vi "Register Events.vi"(8 "error in (no error)":errorcluster, 11 "WebView2 Control in":refnum<class "WebView2 Control.lvclass">) -> (0 "error out":errorcluster, 2 "Events":T1, 3 "WebView2 Control out":refnum<class "WebView2 Control.lvclass">)   [LabVIEW 2020, in "WebView2.lvlib" / "WebView2 Control.lvclass"]
uses:
  WebView2 Control.lvclass
  WebView2 Event Filter Interface/WebView2 Event Filter Interface.lvclass
  E:/Labview/LV 2023/PPL/PPL Builder/Libs/LV-WebView2/Source/Libs/Microsoft.Web.WebView2.Core.dll
  Libs/Microsoft.Web.WebView2.Core.dll
  WebView2 Control.lvclass/WebView2 Control.ctl
  _Raise Nav Complete Event.vi
  _Raise Navigation Starting Event.vi
  _Raise Source Changed Event.vi
  _Raise Document Title Changed.vi
  _Raise StatusBarTextChanged.vi
  _Raise WebMessageReceived.vi
  _Raise WindowCloseRequested.vi
  _Raise Dom Content Loaded.vi
  _Raise New Window Requested.vi
  _Raise Content Loading.vi
  _Raise Context Menu Requested.vi
  _Raise Download Starting.vi
  _Raise Favicon Changed.vi
  _Raise Launching External Uri Scheme.vi
  _Raise Notification Received.vi
  _Raise Permission Requested.vi
  _Raise Save As UI Showing.vi
  _Raise Save File Security Check Starting.vi
  _Raise Script Dialog Opening.vi
  _Raise Server Certificate Error Detected.vi
  _Raise Basic Authentication Requested.vi
  _Raise Client Certificate Requested.vi
  Navigation Event Data.ctl
  Source Changed Event Data.ctl
  Navigation Start Event Data.ctl
  Events.ctl
  New Window Event Data.ctl
  Content Loading Event Data.ctl
  Web Message Received Event Data.ctl
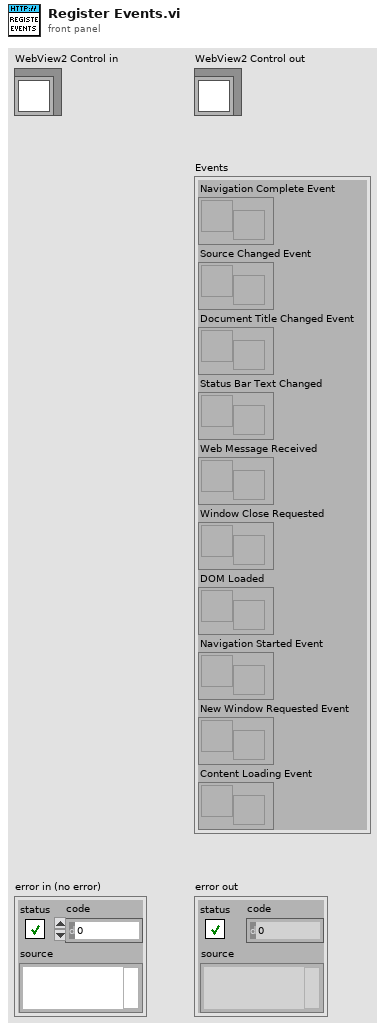
[diagram p1: front panel]
types:
  T1 = typedef "WebView2.lvlib/WebView2 Control.lvclass/Events.ctl" = cluster{"Navigation Complete Event":refnum<user-event>, "Source Changed Event":refnum<user-event>, "Document Title Changed Event":refnum<user-event>, "Status Bar Text Changed":refnum<user-event>, "Web Message Received":refnum<user-event>, "Window Close Requested":refnum<user-event>, "DOM Loaded":refnum<user-event>, "Navigation Started Event":refnum<user-event>, "New Window Requested Event":refnum<user-event>, "Content Loading Event":refnum<user-event>}
  T2 = typedef "WebView2.lvlib/WebView2 Control.lvclass/Res.ctl" = cluster{"WebView2":refnum<k24>, "Webview2 Core":refnum<k24>, "event callback":refnum<k27>, "Environment":refnum<k24>}
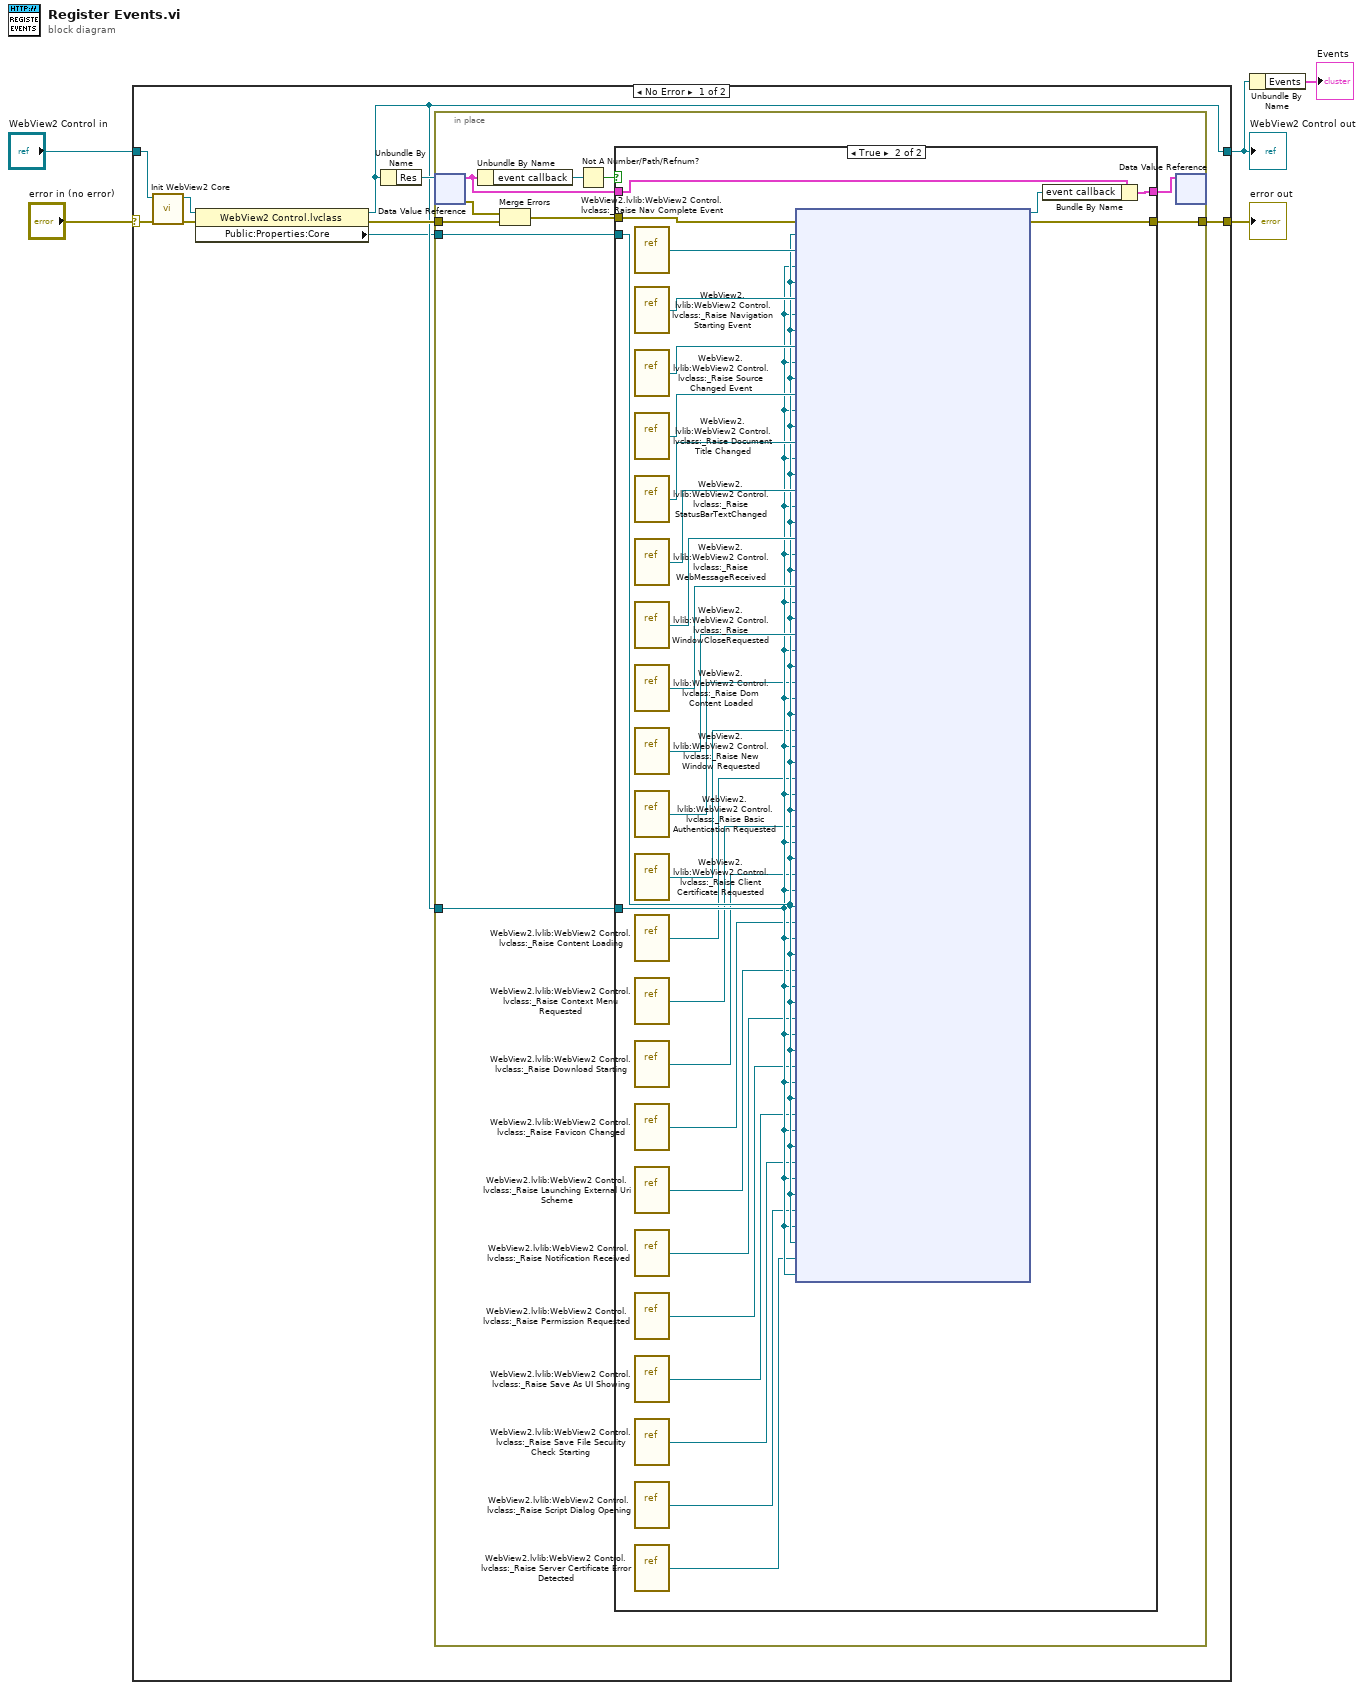
[diagram p0: block diagram]
diagram:
  n1 = case shown="No Error" "error in (no error)" {
    selector: "error in (no error)" -> [w13 w57]
    tunnel: [w7 w56] -> w1
    tunnel: "WebView2 Control in" -> [w14 w56]
    tunnel: [w10 w57] -> w3
    frame No Error {
      n2 = call "Init WebView2 Core.vi"("error in (no error)"=w13, "WebView2"=w14) -> ("error out"=w11:errorcluster, "WebView2.lvlib:WebView2 Control.lvclass"=w8:refnum<class "WebView2 Control.lvclass">)  [unwired: 8 in]
      n3 = property class="WebView2 Control.lvclass"(reference=w8, error in=w11) -> (reference out=w7:refnum<class "WebView2 Control.lvclass">, error out=w9:errorcluster, "Public:Properties:Core"=w6:refnum<k24>)
      n4 = Unbundle By Name(w7) -> ("Res"=w12:refnum<data-value>)
      n5 = in-place {
        in-place-border: w9 -> [w24]
        in-place-border: w7 -> [w21]
        in-place-border: [w20] -> w10
        in-place-border: w6 -> [w15]
        n6 = in-place-dvr #1(w12) -> (w17:T2, w23:errorcluster)
        n7 = Unbundle By Name(w17) -> ("event callback"=w19:refnum<k27>)
        n8 = Merge Errors(w23, w24) -> (w22:errorcluster)
        n9 = Not A Number/Path/Refnum?(number/path/refnum=w19) -> (NaN/Path/Refnum?=w18:bool)
        n10 = case shown="True" w18 {
          tunnel: [w26 w55] -> w20
          tunnel: w22 -> [w26 w51]
          tunnel: w21 -> [_ w40]
          tunnel: w17 -> [w25 w52]
          tunnel: [w25 w53] -> w16
          tunnel: w15 -> [_ w41]
          frame False {
          }
          frame True {
            n11 = vi-ref "WebView2.lvlib:WebView2 Control.lvclass:_Raise Nav Complete Event.vi"() -> (w50:refnum<vi>)
            n12 = vi-ref "WebView2.lvlib:WebView2 Control.lvclass:_Raise Navigation Starting Event.vi"() -> (w49:refnum<vi>)
            n13 = vi-ref "WebView2.lvlib:WebView2 Control.lvclass:_Raise Source Changed Event.vi"() -> (w48:refnum<vi>)
            n14 = vi-ref "WebView2.lvlib:WebView2 Control.lvclass:_Raise Document Title Changed.vi"() -> (w47:refnum<vi>)
            n15 = vi-ref "WebView2.lvlib:WebView2 Control.lvclass:_Raise StatusBarTextChanged.vi"() -> (w46:refnum<vi>)
            n16 = vi-ref "WebView2.lvlib:WebView2 Control.lvclass:_Raise WebMessageReceived.vi"() -> (w45:refnum<vi>)
            n17 = vi-ref "WebView2.lvlib:WebView2 Control.lvclass:_Raise WindowCloseRequested.vi"() -> (w44:refnum<vi>)
            n18 = vi-ref "WebView2.lvlib:WebView2 Control.lvclass:_Raise Dom Content Loaded.vi"() -> (w43:refnum<vi>)
            n19 = vi-ref "WebView2.lvlib:WebView2 Control.lvclass:_Raise New Window Requested.vi"() -> ("vi reference"=w42:refnum<vi>)
            n20 = vi-ref "WebView2.lvlib:WebView2 Control.lvclass:_Raise Basic Authentication Requested.vi"() -> ("vi reference"=w28:refnum<vi>)
            n21 = vi-ref "WebView2.lvlib:WebView2 Control.lvclass:_Raise Client Certificate Requested.vi"() -> ("vi reference"=w27:refnum<vi>)
            n22 = vi-ref "WebView2.lvlib:WebView2 Control.lvclass:_Raise Content Loading.vi"() -> ("vi reference"=w39:refnum<vi>)
            n23 = vi-ref "WebView2.lvlib:WebView2 Control.lvclass:_Raise Context Menu Requested.vi"() -> ("vi reference"=w38:refnum<vi>)
            n24 = vi-ref "WebView2.lvlib:WebView2 Control.lvclass:_Raise Download Starting.vi"() -> ("vi reference"=w37:refnum<vi>)
            n25 = vi-ref "WebView2.lvlib:WebView2 Control.lvclass:_Raise Favicon Changed.vi"() -> ("vi reference"=w36:refnum<vi>)
            n26 = vi-ref "WebView2.lvlib:WebView2 Control.lvclass:_Raise Launching External Uri Scheme.vi"() -> ("vi reference"=w35:refnum<vi>)
            n27 = vi-ref "WebView2.lvlib:WebView2 Control.lvclass:_Raise Notification Received.vi"() -> ("vi reference"=w34:refnum<vi>)
            n28 = vi-ref "WebView2.lvlib:WebView2 Control.lvclass:_Raise Permission Requested.vi"() -> ("vi reference"=w33:refnum<vi>)
            n29 = vi-ref "WebView2.lvlib:WebView2 Control.lvclass:_Raise Save As UI Showing.vi"() -> ("vi reference"=w32:refnum<vi>)
            n30 = vi-ref "WebView2.lvlib:WebView2 Control.lvclass:_Raise Save File Security Check Starting.vi"() -> ("vi reference"=w31:refnum<vi>)
            n31 = vi-ref "WebView2.lvlib:WebView2 Control.lvclass:_Raise Script Dialog Opening.vi"() -> ("vi reference"=w30:refnum<vi>)
            n32 = vi-ref "WebView2.lvlib:WebView2 Control.lvclass:_Raise Server Certificate Error Detected.vi"() -> ("vi reference"=w29:refnum<vi>)
            n33 = node(w51, w41, w50, w40, w41, w49, w40, w41, w48, w40, w41, w47, w40, w41, w46, w40, w41, w45, w40, w41, w44, w40, w41, w43, w40, w41, w42, w40, w41, w28, w40, w41, w27, w40, w41, w39, w40, w41, w38, w40, w41, w37, w40, w41, w36, w40, w41, w35, w40, w41, w34, w40, w41, w33, w40, w41, w32, w40, w41, w31, w40, w41, w30, w40, w41, w29, w40) -> (w54:refnum<k27>, w55:errorcluster)  [unwired: 1 in]
            n34 = Bundle By Name(cluster=w52, "event callback"=w54) -> (w53:T2)
          }
        }
        n35 = in-place-dvr #1(w16) -> ()  [unwired: 2 out]
      }
    }
    frame Error {
    }
  }
  "error out" <- w3
  "WebView2 Control out" <- w1
  n36 = Unbundle By Name(w1) -> ("Events"=→"Events":T1)
